vi "Fibonacci Series.vi"() -> ()   [LabVIEW 2026]
panel:
  out "Fibonacci Series":i64[](array[numeric])
  in  "Number of Terms":i64
  # "Enter the number of terms"
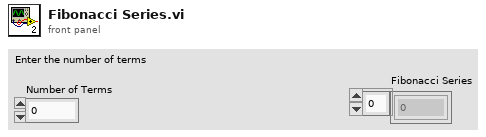
[diagram p1: front panel]
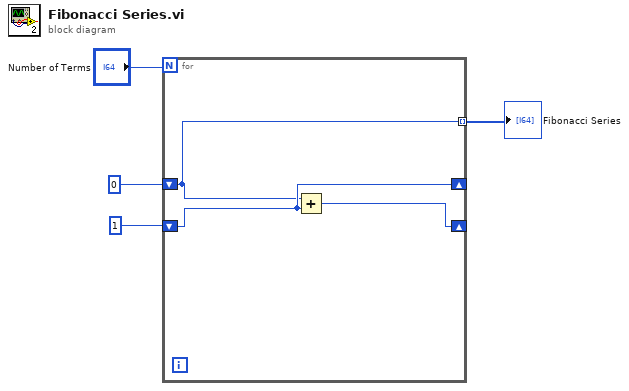
[diagram p0: block diagram]
diagram:
  n1 = for {
    N: "Number of Terms" -> [_]
    shift-right: [w7] -> _
    shift-left: i64 0 -> [w5]
    shift-right: [w6] -> _
    shift-left: i64 1 -> [w7]
    tunnel: [w5] -> w1 mode=indexing
    n2 = Add(x=w5, y=w7) -> (x+y=w6:i64)
  }
  "Fibonacci Series" <- w1
